vi "VIH Project - Control Rule - Apply Default.vi"(8 "default EnumValues":T1, 9 "default ClusterMembers":T1, 10 "default DscrMode":T2, 11 "Control Rules":T3[](array[typedef])) -> (3 "Control Rules out":T3[](array[typedef]))   [LabVIEW 2014]
doc: "::: VI Helpeks :::\nCopyright (c) 2000-2026 Konstantin Shifershteyn. All rights reserved."
uses:
  _VIH HelpGen.llb/VIH HelpGen Typedef - Cluster - Control Rule.ctl
  _VIH HelpGen.llb/VIH HelpGen Typedef - Enum - Description Mode.ctl
  _VIH HelpGen.llb/VIH HelpGen Typedef - Enum - Default,Enable,Disable.ctl
  _VIH HelpGen.llb/VIH HelpGen Typedef - Cluster - Enum Value Info.ctl
panel:
  # "VI Helpeks\nCopyright (c) 2012-2026 Konstantin Shifershteyn"
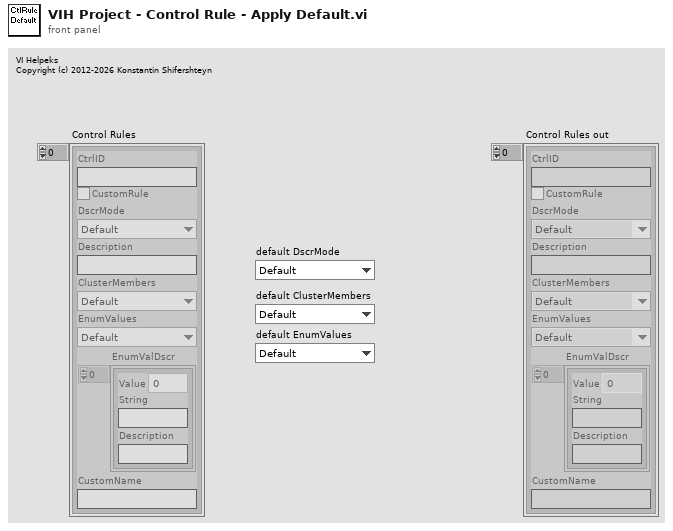
[diagram p1: front panel]
types:
  T1 = typedef "VIH HelpGen Typedef - Enum - Default,Enable,Disable.ctl" = enum16{"Default", "Enable", "Disable"}
  T2 = typedef "VIH HelpGen Typedef - Enum - Description Mode.ctl" = enum16{"Default", "Description", "Description1", "Description2", "Custom", "None"}
  T3 = typedef "VIH HelpGen Typedef - Cluster - Control Rule.ctl" = cluster{"CtrlID":string, "CustomRule":bool, "DscrMode":T2, "Description":string, "ClusterMembers":T1, "EnumValues":T1, "EnumValDscr":T4[], "CustomName":string}
  T4 = typedef "VIH HelpGen Typedef - Cluster - Enum Value Info.ctl" = cluster{"Value":ext, "String":string, "Description":string}
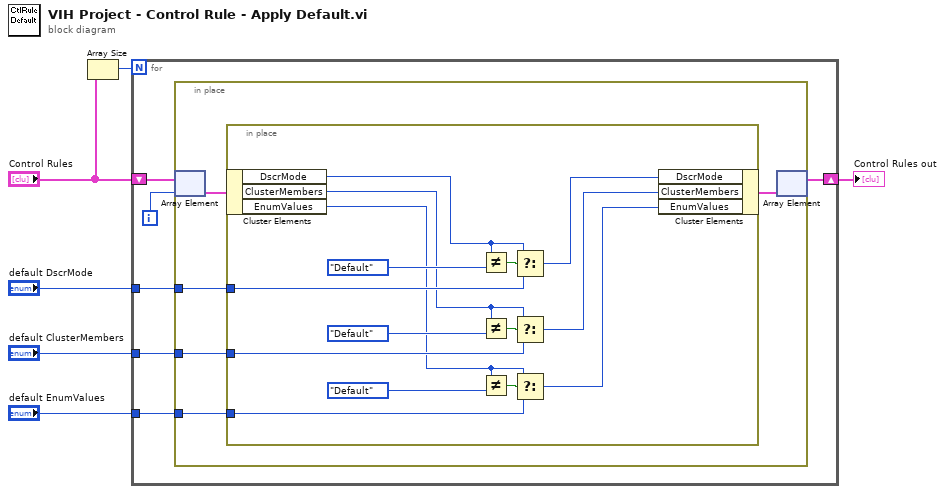
[diagram p0: block diagram]
diagram:
  n1 = Array Size(array="Control Rules") -> (size(s)=w6:i32)
  n2 = for {
    N: w6 -> [_]
    shift-right: [w10] -> w4
    shift-left: "Control Rules" -> [w12]
    tunnel: "default DscrMode" -> [w9]
    tunnel: "default ClusterMembers" -> [w8]
    tunnel: "default EnumValues" -> [w7]
    i -> [w11]
    n3 = in-place {
      in-place-border: w9 -> [w15]
      in-place-border: w8 -> [w14]
      in-place-border: w7 -> [w13]
      n4 = in-place-array #1(w12, w11) -> (w17:T3)
      n5 = in-place {
        in-place-border: w15 -> [w29]
        in-place-border: w14 -> [w24]
        in-place-border: w13 -> [w23]
        n6 = in-place-cluster #2(w17) -> ("DscrMode"=w30:T2, "ClusterMembers"=w21:T1, "EnumValues"=w22:T1)
        n7 = Not Equal?(x=w30, y=VIH_HelpGen_Typedef_-_Enum_-_Description_Mode."Default") -> (x != y?=w31:bool)
        n8 = Not Equal?(x=w21, y=VIH_HelpGen_Typedef_-_Enum_-_Default,Enable,Disable."Default") -> (x != y?=w28:bool)
        n9 = Not Equal?(x=w22, y=VIH_HelpGen_Typedef_-_Enum_-_Default,Enable,Disable."Default") -> (x != y?=w27:bool)
        n10 = Select(t=w30, s=w31, f=w29) -> (s? t:f=w20:T2)
        n11 = Select(t=w21, s=w28, f=w24) -> (s? t:f=w19:T1)
        n12 = Select(t=w22, s=w27, f=w23) -> (s? t:f=w18:T1)
        n13 = in-place-cluster #2("DscrMode"=w20, "ClusterMembers"=w19, "EnumValues"=w18) -> (w16:T3)
      }
      n14 = in-place-array #1(w16) -> (w10:T3[])  [unwired: 1 out]
    }
  }
  "Control Rules out" <- w4
